vi "Save Project.vi"(0 "project reference":refnum<vi>, 5 "measurement core reference":refnum<vi>, 7 "project path":path, 11 "error in":errorcluster) -> (15 "error out":errorcluster)   [LabVIEW 2021, in "Multiple Converter.lvlib"]
uses:
  Multiple Converter.lvlib
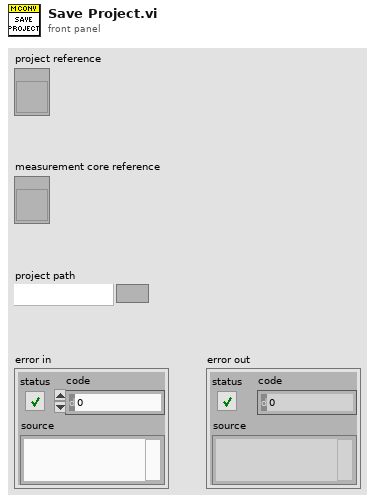
[diagram p1: front panel]
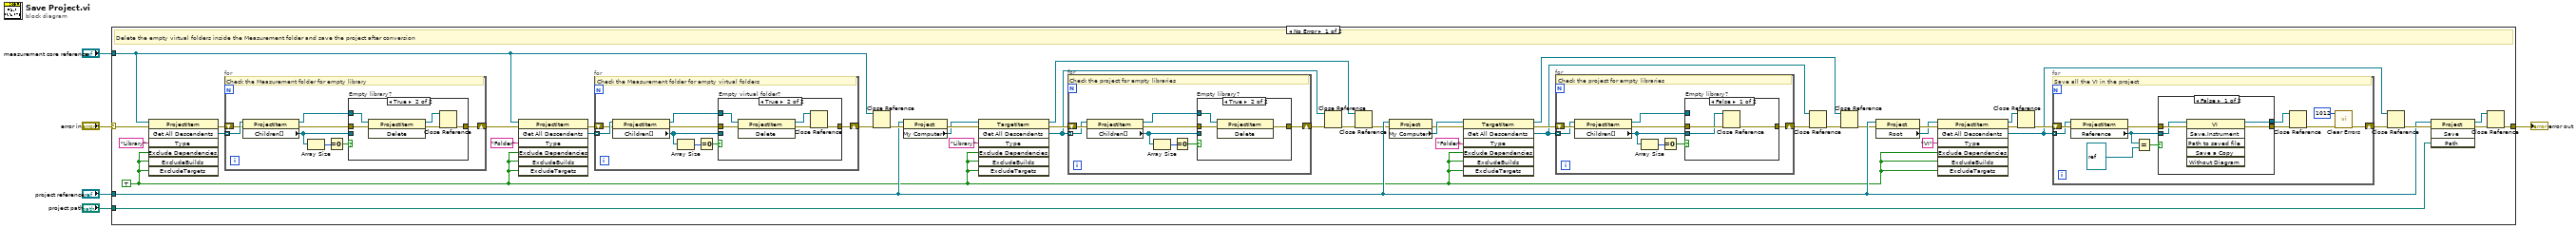
[diagram p0: block diagram]
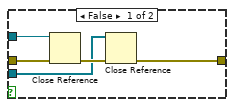
[diagram p2: hidden frame]
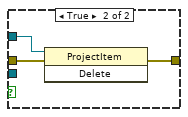
[diagram p3: hidden frame]
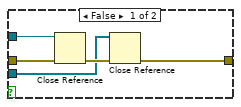
[diagram p4: hidden frame]
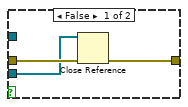
[diagram p5: hidden frame]
diagram:
  n1 = case shown="No Error" "error in" {
    selector: "error in" -> [w15 w131]
    tunnel: [w48 w131] -> w5
    tunnel: "project path" -> [w44 _]
    tunnel: "measurement core reference" -> [w14 _]
    tunnel: "project reference" -> [w24 _]
    frame No Error {
      w8 = TRUE
      # "Delete the empty virtual folders inside the Measurement folder and save the project after conversion"
      n2 = invoke class="ProjectItem" method="Get All Descendents"(reference=w14, error in=w15, "Type"="Library", "Exclude Dependencies"=w8, "ExcludeBuilds"=w8, "ExcludeTargets"=w8) -> (error out=w17:errorcluster, "All Descendents"=w18:refnum<vi>[])  [unwired: 1 in, 5 out]
      n3 = for {
        tunnel: w18 -> [w57] mode=indexing
        shift-right: [w50] -> w7
        shift-left: w17 -> [w56]
        # "Check the Measurement folder for empty library"
        n4 = property class="ProjectItem"(reference=w57, error in=w56) -> (reference out=w52:refnum<vi>, error out=w54:errorcluster, "Children[]"=w51:refnum<vi>[])
        n5 = Array Size(array=w51) -> (size(s)=w55:i32)
        n6 = Equal To 0?(x=w55) -> (x = 0?=w53:bool)
        n7 = case "Empty library?" shown="True" w53 {
          tunnel: w54 -> [w62 w67]
          tunnel: w52 -> [w61 w66]
          tunnel: [w59 w64] -> w50
          tunnel: w51 -> [w58 _]
          frame False {
            n8 = Close Reference(reference=w61, error in (no error)=w62) -> (error out=w60:errorcluster)
            n9 = Close Reference(reference=w58, error in (no error)=w60) -> (error out=w59:errorcluster)
          }
          frame True {
            n10 = invoke class="ProjectItem" method="Delete"(reference=w66, error in=w67) -> (reference out=w63:refnum<vi>, error out=w65:errorcluster)  [unwired: 1 in, 1 out]
            n11 = Close Reference(reference=w63, error in (no error)=w65) -> (error out=w64:errorcluster)
          }
        }
      }
      n12 = invoke class="ProjectItem" method="Get All Descendents"(reference=w14, error in=w7, "Type"="Folder", "Exclude Dependencies"=w8, "ExcludeBuilds"=w8, "ExcludeTargets"=w8) -> (error out=w45:errorcluster, "All Descendents"=w34:refnum<vi>[])  [unwired: 1 in, 5 out]
      n13 = for {
        tunnel: w34 -> [w89] mode=indexing
        shift-right: [w82] -> w6
        shift-left: w45 -> [w88]
        # "Check the Measurement folder for empty virtual folders"
        n14 = property class="ProjectItem"(reference=w89, error in=w88) -> (reference out=w84:refnum<vi>, error out=w86:errorcluster, "Children[]"=w83:refnum<vi>[])
        n15 = Array Size(array=w83) -> (size(s)=w87:i32)
        n16 = Equal To 0?(x=w87) -> (x = 0?=w85:bool)
        n17 = case "Empty virtual folder?" shown="True" w85 {
          tunnel: w86 -> [w94 w99]
          tunnel: w84 -> [w93 w98]
          tunnel: [w91 w96] -> w82
          tunnel: w83 -> [w90 _]
          frame False {
            n18 = Close Reference(reference=w93, error in (no error)=w94) -> (error out=w92:errorcluster)
            n19 = Close Reference(reference=w90, error in (no error)=w92) -> (error out=w91:errorcluster)
          }
          frame True {
            n20 = invoke class="ProjectItem" method="Delete"(reference=w98, error in=w99) -> (reference out=w95:refnum<vi>, error out=w97:errorcluster)  [unwired: 1 in, 1 out]
            n21 = Close Reference(reference=w95, error in (no error)=w97) -> (error out=w96:errorcluster)
          }
        }
      }
      n22 = Close Reference(reference=w14, error in (no error)=w6) -> (error out=w28:errorcluster)
      n23 = property class="Project"(reference=w24, error in=w28) -> (error out=w38:errorcluster, "My Computer"=w29:refnum<vi>)  [unwired: 1 out]
      n24 = invoke class="TargetItem" method="Get All Descendents"(reference=w29, error in=w38, "Type"="Library", "Exclude Dependencies"=w8, "ExcludeBuilds"=w8, "ExcludeTargets"=w8) -> (reference out=w12:refnum<vi>, error out=w36:errorcluster, "All Descendents"=w32:refnum<vi>[])  [unwired: 1 in, 4 out]
      n25 = for {
        shift-right: [w101] -> w33
        shift-left: w36 -> [w107]
        tunnel: w32 -> [w106] mode=indexing
        # "Check the project for empty libraries"
        n26 = property class="ProjectItem"(reference=w106, error in=w107) -> (reference out=w103:refnum<vi>, error out=w102:errorcluster, "Children[]"=w100:refnum<vi>[])
        n27 = Array Size(array=w100) -> (size(s)=w105:i32)
        n28 = Equal To 0?(x=w105) -> (x = 0?=w104:bool)
        n29 = case "Empty library?" shown="True" w104 {
          tunnel: w102 -> [w110 w113]
          tunnel: w103 -> [_ w112]
          tunnel: [w109 w111] -> w101
          tunnel: w100 -> [w108 _]
          frame False {
            n30 = Close Reference(reference=w108, error in (no error)=w110) -> (error out=w109:errorcluster)
          }
          frame True {
            n31 = invoke class="ProjectItem" method="Delete"(reference=w112, error in=w113) -> (error out=w111:errorcluster)  [unwired: 1 in, 2 out]
          }
        }
      }
      n32 = Close Reference(reference=w32, error in (no error)=w33) -> (error out=w23:errorcluster)
      n33 = Close Reference(reference=w12, error in (no error)=w23) -> (error out=w13:errorcluster)
      n34 = property class="Project"(reference=w24, error in=w13) -> (error out=w25:errorcluster, "My Computer"=w27:refnum<vi>)  [unwired: 1 out]
      n35 = invoke class="TargetItem" method="Get All Descendents"(reference=w27, error in=w25, "Type"="Folder", "Exclude Dependencies"=w8, "ExcludeBuilds"=w8, "ExcludeTargets"=w8) -> (reference out=w10:refnum<vi>, error out=w22:errorcluster, "All Descendents"=w19:refnum<vi>[])  [unwired: 1 in, 4 out]
      n36 = for {
        shift-right: [w69] -> w21
        shift-left: w22 -> [w75]
        tunnel: w19 -> [w74] mode=indexing
        # "Check the project for empty libraries"
        n37 = property class="ProjectItem"(reference=w74, error in=w75) -> (reference out=w71:refnum<vi>, error out=w70:errorcluster, "Children[]"=w68:refnum<vi>[])
        n38 = Array Size(array=w68) -> (size(s)=w73:i32)
        n39 = Equal To 0?(x=w73) -> (x = 0?=w72:bool)
        n40 = case "Empty library?" shown="False" w72 {
          tunnel: w70 -> [w78 w81]
          tunnel: w71 -> [_ w80]
          tunnel: [w77 w79] -> w69
          tunnel: w68 -> [w76 _]
          frame False {
            n41 = Close Reference(reference=w76, error in (no error)=w78) -> (error out=w77:errorcluster)
          }
          frame True {
            n42 = invoke class="ProjectItem" method="Delete"(reference=w80, error in=w81) -> (error out=w79:errorcluster)  [unwired: 1 in, 2 out]
          }
        }
      }
      n43 = Close Reference(reference=w19, error in (no error)=w21) -> (error out=w20:errorcluster)
      n44 = Close Reference(reference=w10, error in (no error)=w20) -> (error out=w11:errorcluster)
      n45 = property class="Project"(reference=w24, error in=w11) -> (error out=w43:errorcluster, "Root"=w42:refnum<vi>)  [unwired: 1 out]
      n46 = invoke class="ProjectItem" method="Get All Descendents"(reference=w42, error in=w43, "Type"="VI", "Exclude Dependencies"=w8, "ExcludeBuilds"=w8, "ExcludeTargets"=w8) -> (reference out=w40:refnum<vi>, error out=w41:errorcluster, "All Descendents"=w9:refnum<vi>[])  [unwired: 1 in, 4 out]
      n47 = Close Reference(reference=w40, error in (no error)=w41) -> (error out=w39:errorcluster)
      n48 = for {
        shift-right: [w117] -> w31
        shift-left: w39 -> [w123]
        tunnel: w9 -> [w121] mode=indexing
        # "Save all the VI in the project"
        n49 = property class="ProjectItem"(reference=w121, error in=w123) -> (error out=w122:errorcluster, "Reference"=w118:refnum<vi>)  [unwired: 1 out]
        n50 = Equal?(x=w118, y=refnum<vi> refnum) -> (x = y?=w119:bool)
        n51 = case shown="False" w119 {
          tunnel: [w126 w130] -> w124
          tunnel: w122 -> [w128 w130]
          tunnel: w118 -> [w127 w129]
          tunnel: [w125 w129] -> w114
          frame False {
            n52 = invoke class="VI" method="Save.Instrument"(reference=w127, error in=w128) -> (reference out=w125:refnum<vi>, error out=w126:errorcluster)  [unwired: 4 in, 4 out]
          }
          frame True {
          }
        }
        n53 = Close Reference(reference=w114, error in (no error)=w124) -> (error out=w115:errorcluster)
        n54 = call <vilib>:"Clear Errors.vi"("error in (no error)"=w115, "specific error code to clear (0: all)"=1012) -> ("error out"=w117:errorcluster)  [unwired: 4 in, 1 out]
      }
      n55 = Close Reference(reference=w9, error in (no error)=w31) -> (error out=w30:errorcluster)
      n56 = invoke class="Project" method="Save"(reference=w24, error in=w30, "Path"=w44) -> (reference out=w49:refnum<vi>, error out=w47:errorcluster)  [unwired: 1 in, 2 out]
      n57 = Close Reference(reference=w49, error in (no error)=w47) -> (error out=w48:errorcluster)
    }
    frame Error {
    }
  }
  "error out" <- w5
